vi "D_Check_Disp_IMG.vi"(6 "YPixel":u32, 7 "XPixel":u32, 8 "error in (no error)":errorcluster, 11 "bID":u8) -> (0 "error out":errorcluster, 1 "Read image":picture, 2 "Read array":u8[][](array[numeric]), 3 "bID":u8, 4 "TorF":i32)   [LabVIEW 2015]
uses:
  LabVIEW2018/hpkSLMdaLV.dll
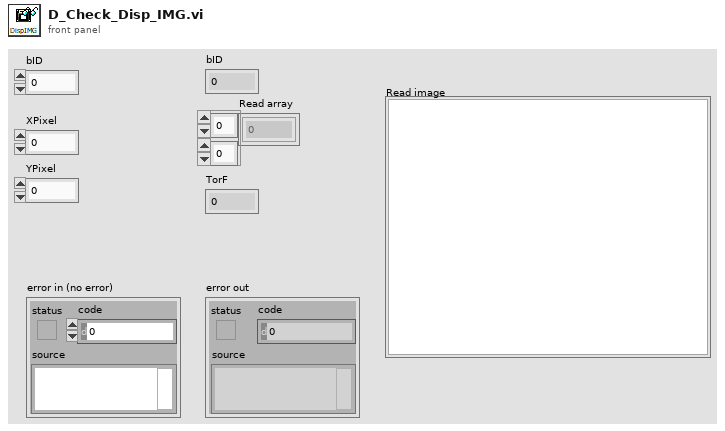
[diagram p1: front panel]
types:
  T1 = typedef "imagedata.ctl" = cluster{"image type":i32, "image depth":i32, "image":u8[], "mask":u8[], "colors":u32[], "Rectangle":cluster{"left":i16, "top":i16, "right":i16, "bottom":i16}}
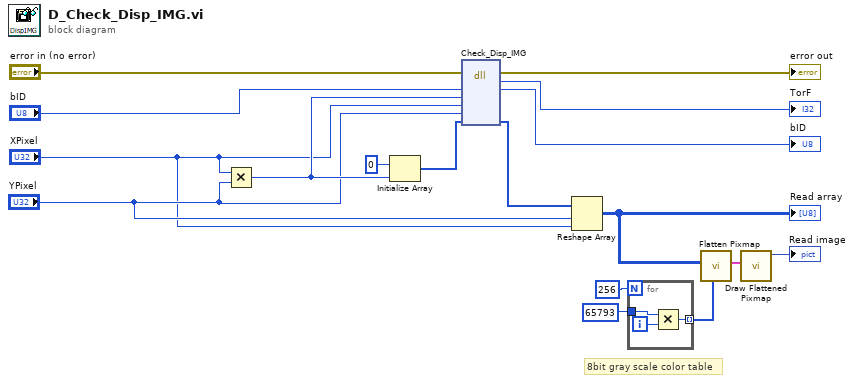
[diagram p0: block diagram]
diagram:
  # "8bit gray scale color table"
  n1 = Multiply(x="XPixel", y="YPixel") -> (x*y=w12:u32)
  n2 = Initialize Array(u8 0, w12) -> (w10:u8[])
  n3 = dll-call lib="C:/Users/hs5921/Desktop/LabVIEW2018/hpkSLMdaLV.dll" fn="Check_Disp_IMG"(error in="error in (no error)", "bID"="bID", "arraySize"=w12, "XPixel"="XPixel", "YPixel"="YPixel", "readArray"=w10) -> (error out=→"error out":errorcluster, "返り値タイプ"=→"TorF":i32, "bID"=→"bID":u8, "readArray"=w9:u8[])  [unwired: 5 in, 1 out]
  n4 = Reshape Array(w9, "YPixel", "XPixel") -> (w2:u8[][])
  "Read array" <- w2
  n5 = for {
    N: 256 -> [_]
    tunnel: 65793 -> [w19]
    tunnel: [w18] -> w6 mode=indexing
    i -> [w20]
    n6 = Multiply(x=w19, y=w20) -> (x*y=w18:i32)
  }
  n7 = call <vilib>:"Flatten Pixmap.vi"("colors"=w6, "8-bit pixmap"=w2) -> ("image data"=w5:T1)  [unwired: 9 in]
  n8 = call <vilib>:"Draw Flattened Pixmap.vi"("image data"=w5) -> ("new picture"=→"Read image":picture)  [unwired: 8 in]
